vi "Shooter_Turret_Motor.vi"(0 "MotorControlDevRef":T3={"DeviceStatus"={"status"=FALSE, "code"=0, "source"=""}, "Type"=enum."PWM", "PWM"={"PWM Channel"=enum."Invalid", "DeadBand"={"Name"="", "maxPositivePwm"=0, "minPositivePwm"=0, "centerPwm"=0, "maxNegativePwm"=0, "minNegativePwm"=0, "angularRange"=0}}, "CAN"={"Device Number"=0, "SetOutput VI Ref"=variant(refnum<vi> refnum), "GetOutput VI Ref"=variant(refnum<vi> refnum), "Enable VI Ref"=variant(refnum<vi> refnum), "Disable VI Ref"=variant(refnum<vi> refnum), "Data"=variant}, "Invert"=FALSE}, 1 "Dt_ Input":dbl, 2 "Pot_Input":dbl, 3 "Pot_Wanted_Value":dbl, 4 "Turret_Clockwise?":bool, 5 "Turret_Counterclockwise?":bool, 6 "TurretParameters":T2={"Scale Positions"={"Forward_StartScale"=0.0, "Reverse_StartScale"=0.0, "Forward_Limit"=0.0, "Reverse_Limit"=0.0}, "Invert?"=FALSE, "PID gains"={"proportional gain (Kc)"=1.0, "integral time (Ti, min)"=0.01, "derivative time (Td, min)"=0.0}} {"PID gains"."derivative time (Td, min)" format="%.3f"; "PID gains"."integral time (Ti, min)" format="%.3f"; "PID gains"."proportional gain (Kc)" format="%.3f"}) -> (20 "Dt_Output":dbl, 21 "TurretPosReached":bool)   [LabVIEW 2016]
uses:
  <vilib>/Rock Robotics/WPI/MotorControl/WPI_MotorControlDeviceRef.ctl
  <vilib>/Rock Robotics/WPI/MotorControl/WPI_MotorControlType.ctl
  <vilib>/Rock Robotics/SystemInterfaces/DIO/FPGA_DIOPWMChannel.ctl
  <vilib>/Rock Robotics/WPI/PWM/WPI_PWMDeadband.ctl
  ArgosLib/Miscellaneous/TypeDefs/MotorLimitPositions_Type.ctl
  <vilib>/addons/control/pid/pid.llb/PID (DBL).vi
  <vilib>/addons/control/pid/NI_PID_pid.lvlib
  ArgosLib/ArgosLib.lvlib
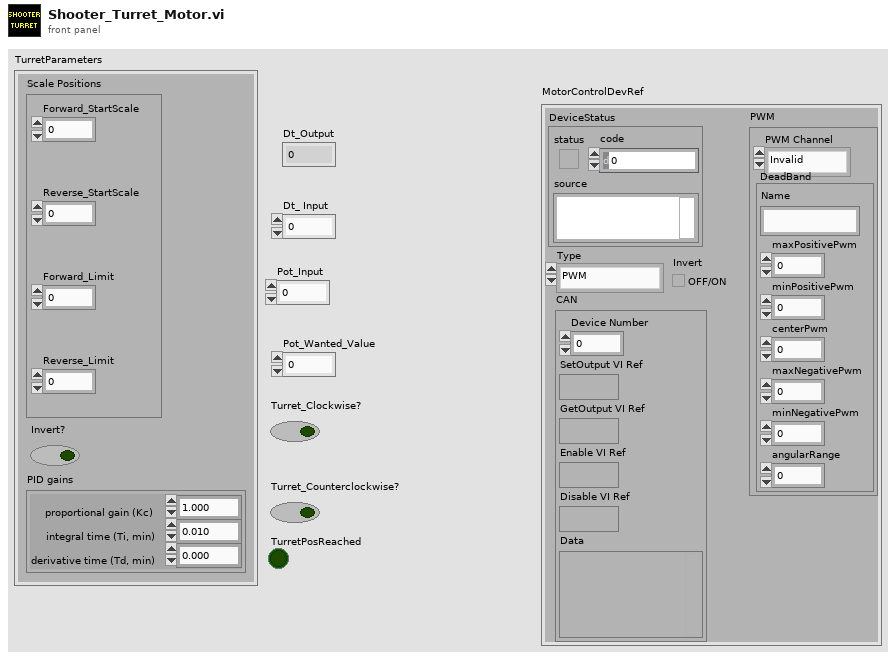
[diagram p1: front panel]
types:
  T1 = typedef "MotorLimitPositions_Type.ctl" = cluster{"Forward_StartScale":dbl, "Reverse_StartScale":dbl, "Forward_Limit":dbl, "Reverse_Limit":dbl}
  T2 = cluster{"Scale Positions":T1, "Invert?":bool, "PID gains":cluster{"proportional gain (Kc)":dbl, "integral time (Ti, min)":dbl, "derivative time (Td, min)":dbl}}
  T3 = typedef "WPI_MotorControlDeviceRef.ctl" = cluster{"DeviceStatus":errorcluster, "Type":T4, "PWM":cluster{"PWM Channel":T5, "DeadBand":T6}, "CAN":cluster{"Device Number":u8, "SetOutput VI Ref":variant, "GetOutput VI Ref":variant, "Enable VI Ref":variant, "Disable VI Ref":variant, "Data":variant}, "Invert":bool}
  T4 = typedef "WPI_MotorControlType.ctl" = enum16{"PWM", "CAN"}
  T5 = typedef "FPGA_DIOPWMChannel.ctl" = enum8{"PWM 0", "PWM 1", "PWM 2", "PWM 3", "PWM 4", "PWM 5", "PWM 6", "PWM 7", "PWM 8", "PWM 9", "PWM MXP 0", "PWM MXP 1", "PWM MXP 2", "PWM MXP 3", "PWM MXP 4", "PWM MXP 5", "PWM MXP 6", "PWM MXP 7", "PWM MXP 8", "PWM MXP 9", "Invalid"}
  T6 = typedef "WPI_PWMDeadband.ctl" = cluster{"Name":string, "maxPositivePwm":i32, "minPositivePwm":i32, "centerPwm":i32, "maxNegativePwm":i32, "minNegativePwm":i32, "angularRange":u16}
  T7 = cluster{"proportional gain (Kc)":dbl, "integral time (Ti, min)":dbl, "derivative time (Td, min)":dbl}
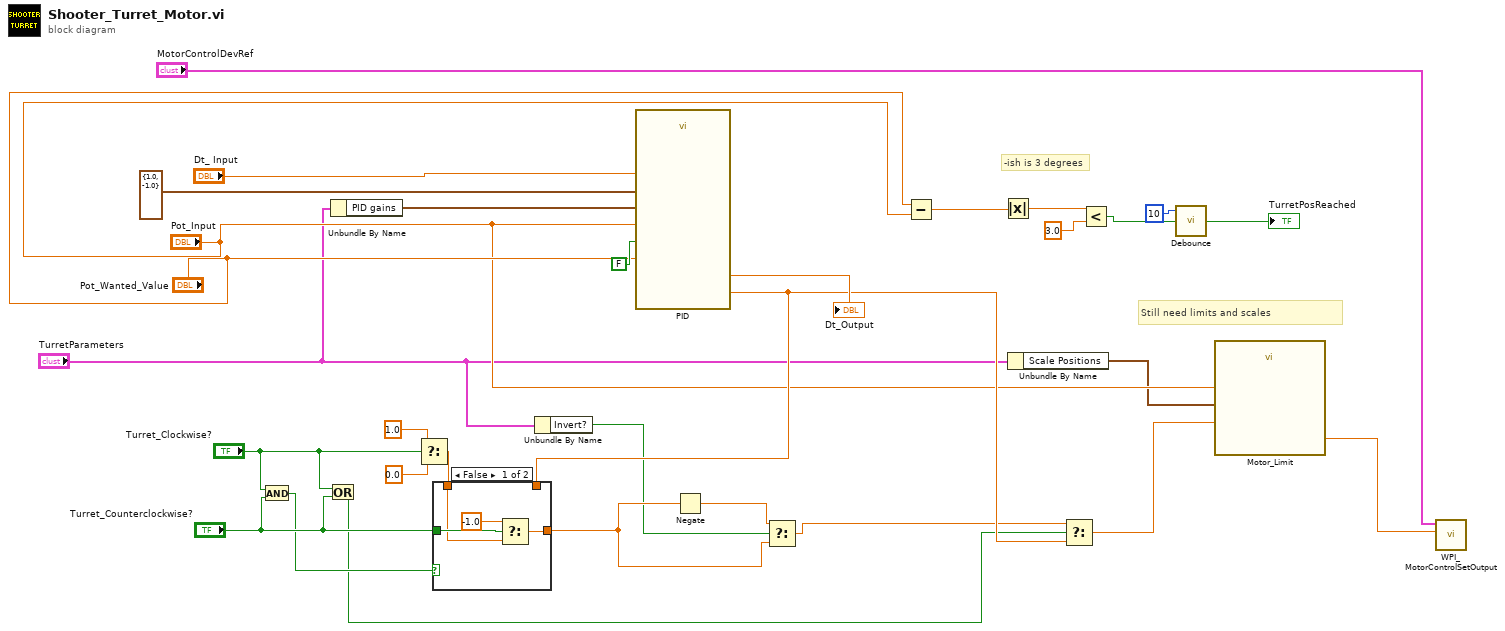
[diagram p0: block diagram]
diagram:
  # "Still need limits and scales"
  # "-ish is 3 degrees"
  n1 = And(x="Turret_Clockwise?", y="Turret_Counterclockwise?") -> (x .and. y?=w17:bool)
  n2 = Or(x="Turret_Clockwise?", y="Turret_Counterclockwise?") -> (x .or. y?=w16:bool)
  n3 = Unbundle By Name("TurretParameters") -> ("PID gains"=w4:T7)
  n4 = Select(t=1.0, s="Turret_Clockwise?", f=0.0) -> (s? t:f=w27:dbl)
  n5 = Unbundle By Name("TurretParameters") -> ("Invert?"=w3:bool)
  n6 = call-poly <vilib>:"PID.vi"("reinitialize? (F)"=FALSE, "output range"=cluster{"output high":dbl, "output low":dbl} {"output high"=1.0, "output low"=-1.0}, "dt (s)"="Dt_ Input", "PID gains"=w4, "process variable"="Pot_Input", "setpoint"="Pot_Wanted_Value") -> ("dt out (s)"=→"Dt_Output":dbl, "output"=w18:dbl)  [unwired: 4 in]
  n7 = case shown="False" w17 {
    tunnel: "Turret_Counterclockwise?" -> [w34 _]
    tunnel: w27 -> [w33 _]
    tunnel: [w31 w35] -> w26
    tunnel: w18 -> [_ w35]
    frame False {
      n8 = Select(t=-1.0, s=w34, f=w33) -> (s? t:f=w31:dbl)
    }
    frame True {
    }
  }
  n9 = Negate(x=w26) -> (-x=w25:dbl)
  n10 = Select(t=w25, s=w3, f=w26) -> (s? t:f=w15:dbl)
  n11 = Subtract(x="Pot_Wanted_Value", y="Pot_Input") -> (x-y=w14:dbl)
  n12 = Absolute Value(x=w14) -> (abs(x)=w13:dbl)
  n13 = Unbundle By Name("TurretParameters") -> ("Scale Positions"=w1:T1)
  n14 = Select(t=w15, s=w16, f=w18) -> (s? t:f=w6:dbl)
  n15 = Less?(x=w13, y=3.0) -> (x < y?=w10:bool)
  n16 = call "Debounce.vi"("Input"=w10, "Num samples"=10) -> ("Output"=→"TurretPosReached":bool)  [unwired: 1 in]
  n17 = call "Motor_Limit.vi"("Current_Pos"="Pot_Input", "Motor_Speed"=w6, "Scale Positions"=w1) -> ("New_Motor_Speed"=w7:dbl)  [unwired: 15 in, 1 out]
  n18 = call <vilib>:"WPI_MotorControlSetOutput.vi"("Output"=w7, "MotorControlDevRef"="MotorControlDevRef") -> ()  [unwired: 7 in, 3 out]
